vi "Global Log To String.vi"(10 "Log":T1) -> (3 "Log String":string)   [LabVIEW 2017, in "Communicable State Machine.lvlib"]
doc: "Converts global log data clusters to strings.\n\n-- <b>Controls</b> --\n- <b>Log</b>: Global log data cluster.\n\n-- <b>Indicators</b> --\n- <b>Log String</b>: Global log string."
uses:
  Communicable State Machine.lvlib
  _Support/Typedef/_CSM_GlobalLog_MSG.ctl
  _Support/Typedef/_CSM_Response Source Message.ctl
  _Support/Typedef/_CSM_GlobalLog_MSG_TYPE.ctl
  _Shared/CSM Shared.lvlib
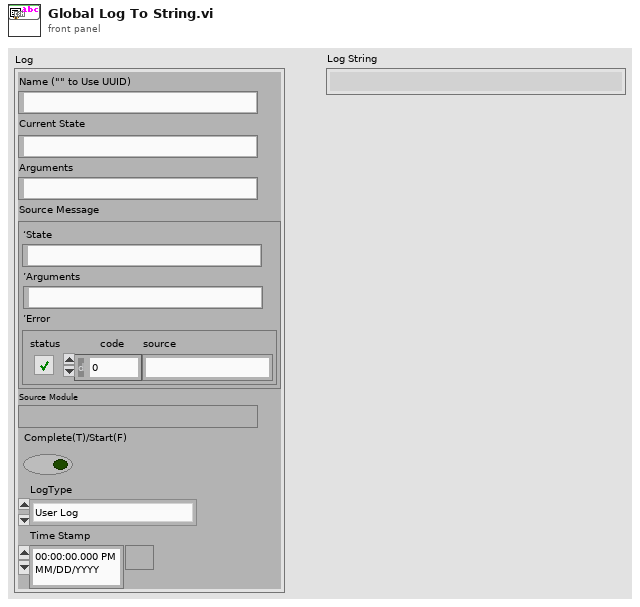
[diagram p1: front panel]
types:
  T1 = typedef "Communicable State Machine.lvlib/_CSM_GlobalLog_MSG.ctl" = cluster{"Name (\"\" to Use UUID)":string, "Current State":string, "Arguments":string, "Source Message":T2, "Source Module":string, "Complete(T)/Start(F)":bool, "LogType":T3, "Time Stamp":timestamp}
  T2 = typedef "Communicable State Machine.lvlib/_CSM_Response Source Message.ctl" = cluster{"‘State":string, "’Arguments":string, "’Error":errorcluster}
  T3 = typedef "Communicable State Machine.lvlib/_CSM_GlobalLog_MSG_TYPE.ctl" = enum16{"User Log", "State Change", "Status", "Interrupt", "Register", "Unregister", "Error Log", "Module Created", "Module Destroyed", "Async Message", "No-Rep Async Message", "Sync Message"}
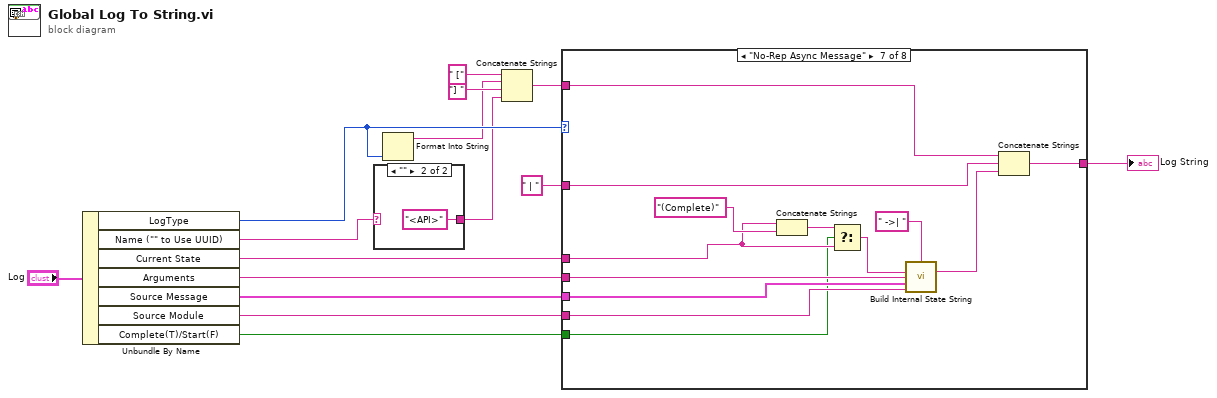
[diagram p0: block diagram]
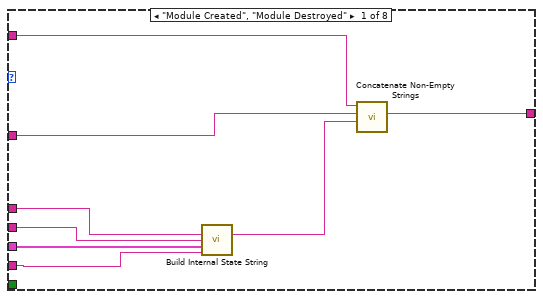
[diagram p3: hidden frame]
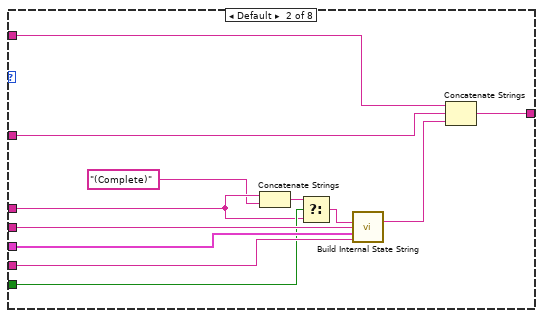
[diagram p4: hidden frame]
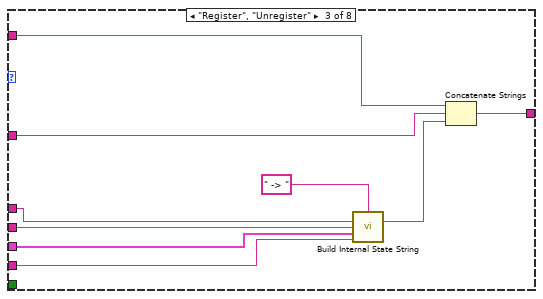
[diagram p5: hidden frame]
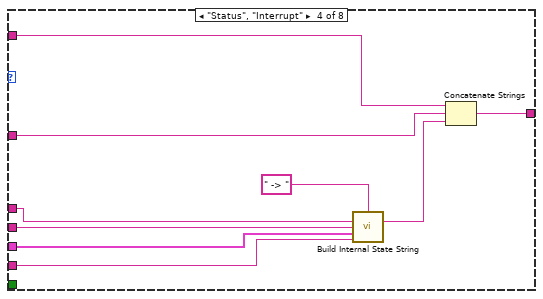
[diagram p6: hidden frame]
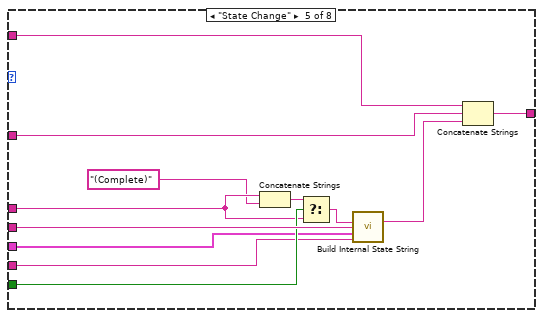
[diagram p7: hidden frame]
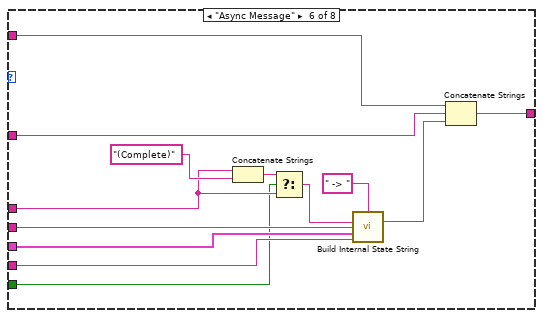
[diagram p8: hidden frame]
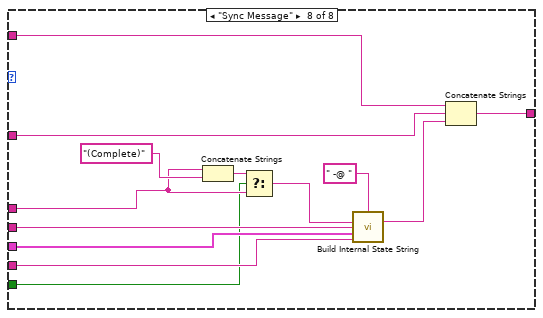
[diagram p9: hidden frame]
diagram:
  n1 = Unbundle By Name("Log") -> ("LogType"=w13:T3, "Name (\"\" to Use UUID)"=w2:string, "Current State"=w8:string, "Arguments"=w11:string, "Source Message"=w10:T2, "Source Module"=w9:string, "Complete(T)/Start(F)"=w7:bool)
  n2 = case shown="\"\"" w2 {
    selector: w2 -> [w16 _]
    tunnel: [w16 "<API>"] -> w1
    frame Default {
    }
    frame "" {
    }
  }
  n3 = Format Into String(w13) -> (resulting string=w4:string)  [unwired: 3 in, 1 out]
  n4 = Concatenate Strings(" [" ("string"), w4, "] " ("string"), w1) -> (w3:string)
  n5 = case shown="\"No-Rep Async Message\"" w13 {
    tunnel: [w24 w37 w46 w55 w67 w80 w93 w106] -> w14
    tunnel: " | " ("string") -> [w25 w36 w45 w54 w66 w79 w92 w105]
    tunnel: w11 -> [w19 w33 w44 w53 w63 w78 w91 w104]
    tunnel: w10 -> [w21 w32 w43 w52 w57 w77 w90 w103]
    tunnel: w9 -> [w18 w31 w42 w51 w56 w76 w89 w102]
    tunnel: w8 -> [w20 w29 w41 w50 w61 w70 w83 w96]
    tunnel: w7 -> [_ w30 _ _ w62 w68 w81 w94]
    tunnel: w3 -> [w23 w26 w39 w48 w58 w74 w87 w100]
    frame "Module Created", "Module Destroyed" {
      n6 = call "Build Internal State String.vi"("State"=w20, "Arguments (\"\")"=w19, "Additional Information"=w21, "Source (\"\")"=w18) -> ("State With Arguments"=w22:string)  [unwired: 11 in]
      n7 = call "Concatenate Non-Empty Strings.vi"("String2"=w22, "Seperator(Carriage Return)"=w25, "String1"=w23) -> ("Result String"=w24:string)  [unwired: 5 in]
    }
    frame Default {
      n8 = Concatenate Strings(w29, "(Complete)" ("string")) -> (w35:string)
      n9 = Select(t=w35, s=w30, f=w29) -> (s? t:f=w34:string)
      n10 = call "Build Internal State String.vi"("State"=w34, "Arguments (\"\")"=w33, "Additional Information"=w32, "Source (\"\")"=w31) -> ("State With Arguments"=w27:string)  [unwired: 11 in]
      n11 = Concatenate Strings(w26, w36, w27) -> (w37:string)
    }
    frame "Register", "Unregister" {
      n12 = call "Build Internal State String.vi"("Seperator(<-)"=" -> ", "State"=w41, "Arguments (\"\")"=w44, "Additional Information"=w43, "Source (\"\")"=w42) -> ("State With Arguments"=w40:string)  [unwired: 10 in]
      n13 = Concatenate Strings(w39, w45, w40) -> (w46:string)
    }
    frame "Status", "Interrupt" {
      n14 = call "Build Internal State String.vi"("Seperator(<-)"=" -> ", "State"=w50, "Arguments (\"\")"=w53, "Additional Information"=w52, "Source (\"\")"=w51) -> ("State With Arguments"=w49:string)  [unwired: 10 in]
      n15 = Concatenate Strings(w48, w54, w49) -> (w55:string)
    }
    frame "State Change" {
      n16 = Concatenate Strings(w61, "(Complete)" ("string")) -> (w65:string)
      n17 = Select(t=w65, s=w62, f=w61) -> (s? t:f=w64:string)
      n18 = call "Build Internal State String.vi"("State"=w64, "Arguments (\"\")"=w63, "Additional Information"=w57, "Source (\"\")"=w56) -> ("State With Arguments"=w59:string)  [unwired: 11 in]
      n19 = Concatenate Strings(w58, w66, w59) -> (w67:string)
    }
    frame "Async Message" {
      n20 = Concatenate Strings(w70, "(Complete)" ("string")) -> (w72:string)
      n21 = Select(t=w72, s=w68, f=w70) -> (s? t:f=w69:string)
      n22 = call "Build Internal State String.vi"("Seperator(<-)"=" -> ", "State"=w69, "Arguments (\"\")"=w78, "Additional Information"=w77, "Source (\"\")"=w76) -> ("State With Arguments"=w75:string)  [unwired: 10 in]
      n23 = Concatenate Strings(w74, w79, w75) -> (w80:string)
    }
    frame "No-Rep Async Message" {
      n24 = Concatenate Strings(w83, "(Complete)" ("string")) -> (w85:string)
      n25 = Select(t=w85, s=w81, f=w83) -> (s? t:f=w82:string)
      n26 = call "Build Internal State String.vi"("Seperator(<-)"=" ->| ", "State"=w82, "Arguments (\"\")"=w91, "Additional Information"=w90, "Source (\"\")"=w89) -> ("State With Arguments"=w88:string)  [unwired: 10 in]
      n27 = Concatenate Strings(w87, w92, w88) -> (w93:string)
    }
    frame "Sync Message" {
      n28 = Concatenate Strings(w96, "(Complete)" ("string")) -> (w98:string)
      n29 = Select(t=w98, s=w94, f=w96) -> (s? t:f=w95:string)
      n30 = call "Build Internal State String.vi"("Seperator(<-)"=" -@ ", "State"=w95, "Arguments (\"\")"=w104, "Additional Information"=w103, "Source (\"\")"=w102) -> ("State With Arguments"=w101:string)  [unwired: 10 in]
      n31 = Concatenate Strings(w100, w105, w101) -> (w106:string)
    }
  }
  "Log String" <- w14
